vi "Get PLC Type.vi"(9 "error in (no error)":errorcluster, 10 ".NET AdsDataType in":refnum<k24>) -> (1 "error out":errorcluster, 2 ".NET AdsDataType":refnum<k24>, 3 "PLC Type":T1)   [LabVIEW 2018, in "TwinCAT ADS.lvclass"]
uses:
  TwinCAT ADS.lvclass
  TwinCAT.Ads
  Controls/PLC Type.ctl
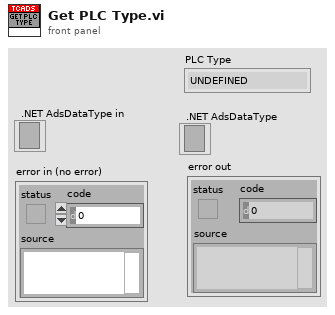
[diagram p1: front panel]
types:
  T1 = typedef "TwinCAT ADS.lvclass/PLC Type.ctl" = enum16{"UNDEFINED", "INT", "DINT", "REAL", "LREAL", "SINT", "BYTE", "UINT", "UDINT", "LINT", "ULINT", "STRING", "WSTRING", "BOOL", "TIME", "LTIME", "DATE", "DT", "TOD", "ARRAY", "JAGGED ARRAY", "STRUCT", "FUNCTION BLOCK", "POINTER", "USER DEFINED"}
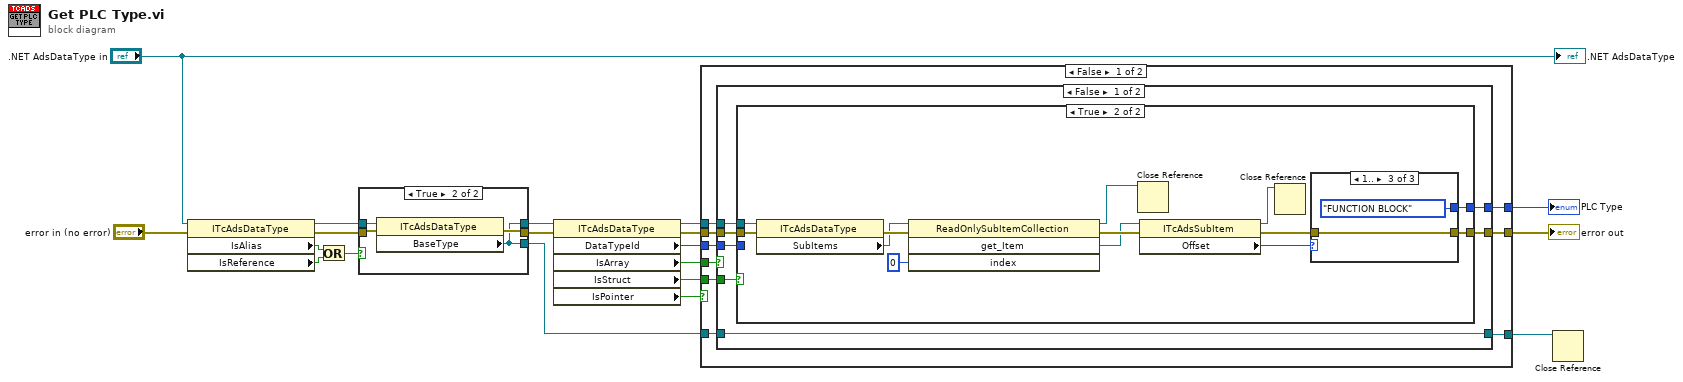
[diagram p0: block diagram]
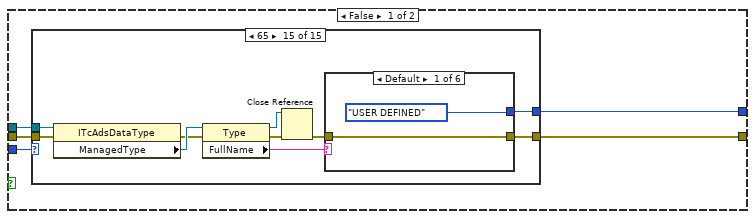
[diagram p3: hidden frame]
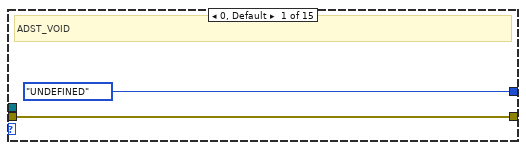
[diagram p4: hidden frame]
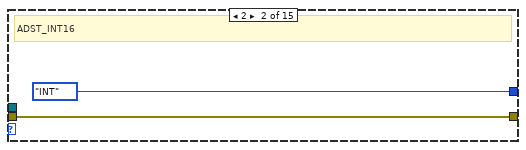
[diagram p5: hidden frame]
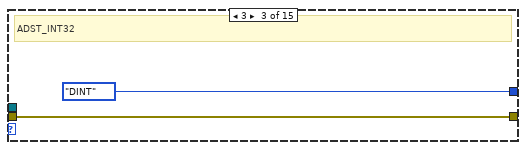
[diagram p6: hidden frame]
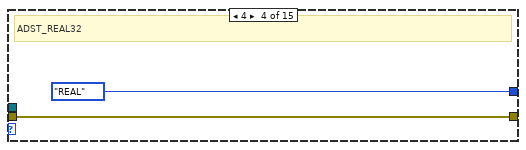
[diagram p7: hidden frame]
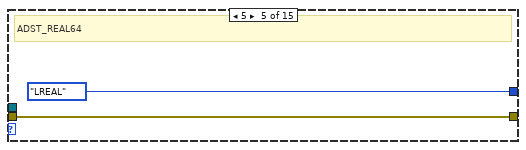
[diagram p8: hidden frame]
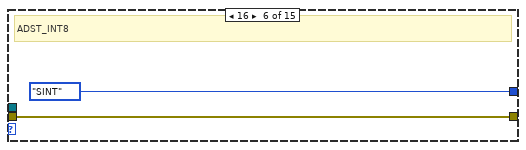
[diagram p9: hidden frame]
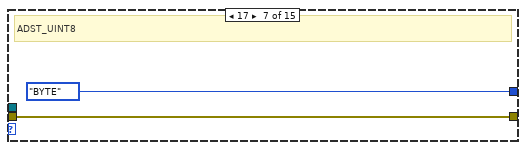
[diagram p10: hidden frame]
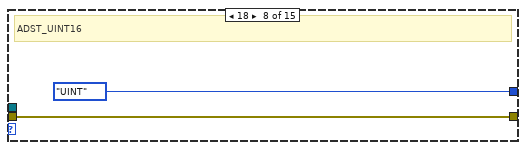
[diagram p11: hidden frame]
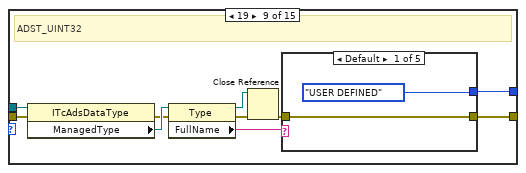
[diagram p12: hidden frame]
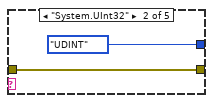
[diagram p13: hidden frame]
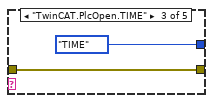
[diagram p14: hidden frame]
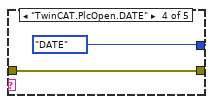
[diagram p15: hidden frame]
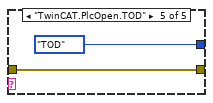
[diagram p16: hidden frame]
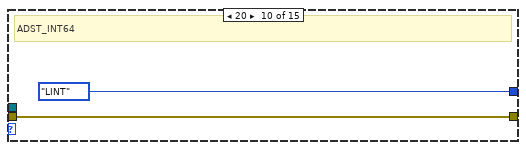
[diagram p17: hidden frame]
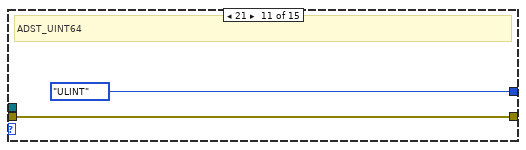
[diagram p18: hidden frame]
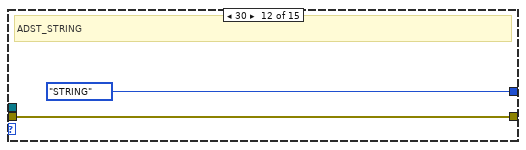
[diagram p19: hidden frame]
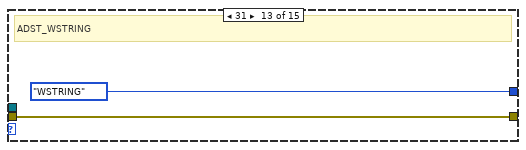
[diagram p20: hidden frame]
diagram:
  n1 = property class="ITcAdsDataType"(reference=".NET AdsDataType in", error in="error in (no error)") -> (reference out=w8:refnum<k24>, error out=w4:errorcluster, "IsAlias"=w6:bool, "IsReference"=w5:bool)
  n2 = Or(x=w6, y=w5) -> (x .or. y?=w7:bool)
  n3 = case shown="True" w7 {
    tunnel: w8 -> [w21 w25]
    tunnel: w4 -> [w20 w24]
    tunnel: [w21 w22] -> w3
    tunnel: [w20 w23] -> w2
    tunnel: [_ w22] -> w1
    frame False {
    }
    frame True {
      n4 = property class="ITcAdsDataType"(reference=w25, error in=w24) -> (error out=w23:errorcluster, "BaseType"=w22:refnum<k24>)  [unwired: 1 out]
    }
  }
  n5 = property class="ITcAdsDataType"(reference=w3, error in=w2) -> (reference out=w17:refnum<k24>, error out=w18:errorcluster, "DataTypeId"=w19:i32, "IsArray"=w14:bool, "IsStruct"=w13:bool, "IsPointer"=w9:bool)
  n6 = case shown="False" w9 {
    tunnel: w19 -> [w34 _]
    tunnel: w18 -> [w33 w143]
    tunnel: w17 -> [w32 _]
    tunnel: [w31 PLC_Type."POINTER" ("PLC Type")] -> w16
    tunnel: [w30 w143] -> w15
    tunnel: w14 -> [w29 _]
    tunnel: w13 -> [w28 _]
    tunnel: w1 -> [w27 w144]
    tunnel: [w26 w144] -> w12
    frame False {
      n7 = case shown="False" w29 {
        tunnel: w34 -> [w41 _]
        tunnel: w33 -> [w40 w141]
        tunnel: w32 -> [w39 w140]
        tunnel: [w38 w137] -> w31
        tunnel: [w37 w139] -> w30
        tunnel: w28 -> [w36 _]
        tunnel: w27 -> [w35 w134]
        tunnel: [w35 w134] -> w26
        frame False {
          n8 = case shown="True" w36 {
            tunnel: w41 -> [w46 _]
            tunnel: w40 -> [w45 w127]
            tunnel: w39 -> [w44 w126]
            tunnel: [w43 w116] -> w38
            tunnel: [w42 w117] -> w37
            frame False {
              n9 = case shown="65" w46 {
                tunnel: [PLC_Type."UNDEFINED" ("PLC Type") PLC_Type."INT" ("PLC Type") PLC_Type."DINT" ("PLC Type") PLC_Type."REAL" ("PLC Type") PLC_Type."LREAL" ("PLC Type") PLC_Type."SINT" ("PLC Type") PLC_Type."BYTE" ("PLC Type") PLC_Type."UINT" ("PLC Type") w69 PLC_Type."LINT" ("PLC Type") PLC_Type."ULINT" ("PLC Type") PLC_Type."STRING" ("PLC Type") PLC_Type."WSTRING" ("PLC Type") PLC_Type."BOOL" ("PLC Type") w94] -> w43
                tunnel: w45 -> [w48 w50 w52 w54 w56 w58 w60 w62 w65 w84 w86 w88 w89 w92 w99]
                tunnel: [w48 w50 w52 w54 w56 w58 w60 w62 w72 w84 w86 w88 w89 w92 w93] -> w42
                tunnel: w44 -> [_ _ _ _ _ _ _ _ w64 _ _ _ _ _ w98]
                frame 0, Default {
                  # "ADST_VOID"
                }
                frame 2 {
                  # "ADST_INT16"
                }
                frame 3 {
                  # "ADST_INT32"
                }
                frame 4 {
                  # "ADST_REAL32"
                }
                frame 5 {
                  # "ADST_REAL64"
                }
                frame 16 {
                  # "ADST_INT8"
                }
                frame 17 {
                  # "ADST_UINT8"
                }
                frame 18 {
                  # "ADST_UINT16"
                }
                frame 19 {
                  # "ADST_UINT32"
                  n10 = property class="ITcAdsDataType"(reference=w64, error in=w65) -> (error out=w63:errorcluster, "ManagedType"=w71:refnum<k24>)  [unwired: 1 out]
                  n11 = property class="Type"(reference=w71, error in=w63) -> (reference out=w66:refnum<k24>, error out=w68:errorcluster, "FullName"=w70:string)
                  n12 = Close Reference(reference=w66, error in (no error)=w68) -> (error out=w67:errorcluster)
                  n13 = case shown="Default" w70 {
                    tunnel: [w74 w76 w78 w80 w82] -> w72
                    tunnel: w67 -> [w74 w76 w78 w80 w82]
                    tunnel: [PLC_Type."USER DEFINED" ("PLC Type") PLC_Type."UDINT" ("PLC Type") PLC_Type."TIME" ("PLC Type") PLC_Type."DATE" ("PLC Type") PLC_Type."TOD" ("PLC Type")] -> w69
                    frame Default {
                    }
                    frame "System.UInt32" {
                    }
                    frame "TwinCAT.PlcOpen.TIME" {
                    }
                    frame "TwinCAT.PlcOpen.DATE" {
                    }
                    frame "TwinCAT.PlcOpen.TOD" {
                    }
                  }
                }
                frame 20 {
                  # "ADST_INT64"
                }
                frame 21 {
                  # "ADST_UINT64"
                }
                frame 30 {
                  # "ADST_STRING"
                }
                frame 31 {
                  # "ADST_WSTRING"
                }
                frame 33 {
                  # "ADST_BIT"
                }
                frame 65 {
                  n14 = property class="ITcAdsDataType"(reference=w98, error in=w99) -> (error out=w97:errorcluster, "ManagedType"=w102:refnum<k24>)  [unwired: 1 out]
                  n15 = property class="Type"(reference=w102, error in=w97) -> (reference out=w100:refnum<k24>, error out=w101:errorcluster, "FullName"=w96:string)
                  n16 = Close Reference(reference=w100, error in (no error)=w101) -> (error out=w95:errorcluster)
                  n17 = case shown="Default" w96 {
                    tunnel: [w104 w106 w108 w110 w112 w114] -> w93
                    tunnel: w95 -> [w104 w106 w108 w110 w112 w114]
                    tunnel: [PLC_Type."USER DEFINED" ("PLC Type") PLC_Type."TIME" ("PLC Type") PLC_Type."LTIME" ("PLC Type") PLC_Type."DATE" ("PLC Type") PLC_Type."DT" ("PLC Type") PLC_Type."TOD" ("PLC Type")] -> w94
                    frame Default {
                    }
                    frame "TwinCAT.PlcOpen.TIME" {
                    }
                    frame "TwinCAT.PlcOpen.LTIME" {
                    }
                    frame "TwinCAT.PlcOpen.DATE" {
                    }
                    frame "TwinCAT.PlcOpen.DT" {
                    }
                    frame "TwinCAT.PlcOpen.TOD" {
                    }
                  }
                }
              }
            }
            frame True {
              n18 = property class="ITcAdsDataType"(reference=w126, error in=w127) -> (error out=w125:errorcluster, "SubItems"=w124:refnum<k24>)  [unwired: 1 out]
              n19 = invoke class="ReadOnlySubItemCollection" method="get_Item"(reference=w124, error in=w125, "index"=0) -> (reference out=w120:refnum<k24>, error out=w122:errorcluster, "get_Item"=w121:refnum<k24>)  [unwired: 1 in, 1 out]
              n20 = Close Reference(reference=w120) -> ()  [unwired: 1 in, 1 out]
              n21 = property class="ITcAdsSubItem"(reference=w121, error in=w122) -> (reference out=w115:refnum<k24>, error out=w118:errorcluster, "Offset"=w119:i32)
              n22 = Close Reference(reference=w115) -> ()  [unwired: 1 in, 1 out]
              n23 = case shown="1.." w119 {
                tunnel: w118 -> [w129 w131 w133]
                tunnel: [w129 w131 w133] -> w117
                tunnel: [PLC_Type."UNDEFINED" ("PLC Type") PLC_Type."STRUCT" ("PLC Type") PLC_Type."FUNCTION BLOCK" ("PLC Type")] -> w116
                frame ..-1 {
                }
                frame 0 {
                }
                frame 1.. {
                }
              }
            }
          }
        }
        frame True {
          n24 = property class="ITcAdsDataType"(reference=w140, error in=w141) -> (error out=w139:errorcluster, "IsJaggedArray"=w138:bool)  [unwired: 1 out]
          n25 = Select(t=PLC_Type."JAGGED ARRAY" ("PLC Type"), s=w138, f=PLC_Type."ARRAY" ("PLC Type")) -> (s? t:f=w137:T1)
        }
      }
    }
    frame True {
    }
  }
  "error out" <- w15
  "PLC Type" <- w16
  n26 = Close Reference(reference=w12) -> ()  [unwired: 1 in, 1 out]
  ".NET AdsDataType" <- ".NET AdsDataType in"
